vi "macro_LinearFilter_ExecuteAVG.vi"   [LabVIEW 2019, in "Trajectory_Library.lvlib"]
uses:
  Trajectory_Library.lvlib
  LinearFilter_MovingAvg_Execute.vi
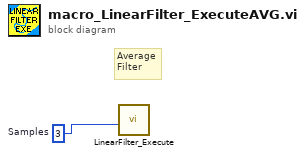
[diagram p0: block diagram]
diagram:
  w1 = 3  # Samples
  # "Average\nFilter"
  n1 = call-poly "LinearFilter_Execute.vi"("Samples"=w1) -> ()  [unwired: 10 in, 1 out]
